vi "RemoteVI Complex Fixture Prep Panel.vi"(0 "path":path, 11 "error in":errorcluster) -> (15 "error out":errorcluster)   [LabVIEW 2020]
doc: "Build helper of RemoteVI Complex Fixture.vi (AIXML cannot create panes or splitter bars). Edits the VI at path - a COPY of NI's example Resizable Panel with Splitter Bars.vi - so that its panel keeps its three panes and its two splitter bars but holds no control and no decoration: every control and every decoration (the example's instructions) is deleted, and the VI is saved. Its diagram is left for lvai_graft_diagram (replaceDiagram) to discard."
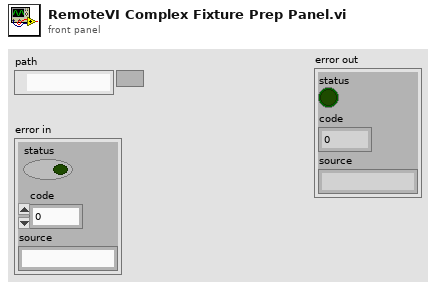
[diagram p1: front panel]
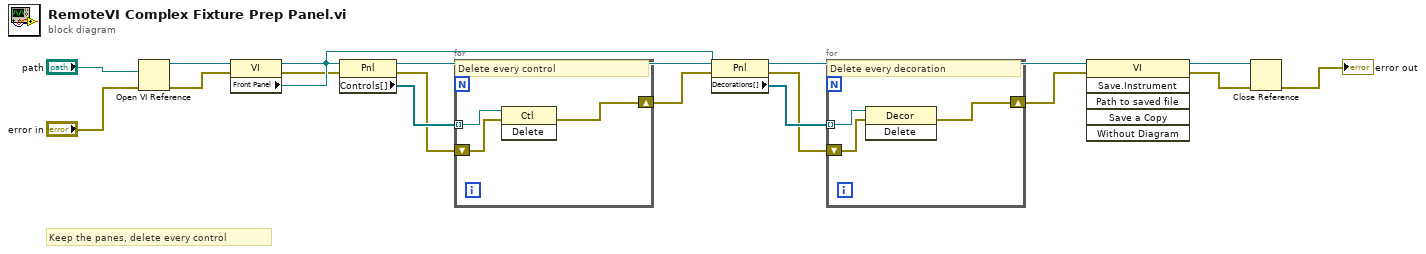
[diagram p0: block diagram]
diagram:
  # "Keep the panes, delete every control"
  n1 = Open VI Reference(vi path="path", error in (no error)="error in") -> (vi reference=w3:refnum<vi>, error out=w4:errorcluster)  [unwired: 4 in]
  n2 = property class="VI"(reference=w3, error in=w4) -> (reference out=w5:refnum<vi>, error out=w6:errorcluster, "Front Panel"=w7:refnum<vi>)
  n3 = property class="Pnl"(reference=w7, error in=w6) -> (error out=w8:errorcluster, "Controls[]"=w9:refnum<vi>[])  [unwired: 1 out]
  n4 = for {
    tunnel: w9 -> [w17] mode=indexing
    shift-right: [w19] -> w10
    shift-left: w8 -> [w18]
    # "Delete every control"
    n5 = invoke class="Ctl" method="Delete"(reference=w17, error in=w18) -> (error out=w19:errorcluster)  [unwired: 1 in, 2 out]
  }
  n6 = property class="Pnl"(reference=w7, error in=w10) -> (error out=w11:errorcluster, "Decorations[]"=w12:refnum<vi>[])  [unwired: 1 out]
  n7 = for {
    tunnel: w12 -> [w20] mode=indexing
    shift-right: [w22] -> w13
    shift-left: w11 -> [w21]
    # "Delete every decoration"
    n8 = invoke class="Decor" method="Delete"(reference=w20, error in=w21) -> (error out=w22:errorcluster)  [unwired: 1 in, 2 out]
  }
  n9 = invoke class="VI" method="Save.Instrument"(reference=w5, error in=w13) -> (reference out=w14:refnum<vi>, error out=w15:errorcluster)  [unwired: 4 in, 4 out]
  n10 = Close Reference(reference=w14, error in (no error)=w15) -> (error out=→"error out":errorcluster)
